vi "table line to assembly.vi"(11 "ItemNames":string[](array[string])) -> (3 "assembly definition":T1)   [LabVIEW 2013, in "EthernetIP editor node.lvclass"]
uses:
  EthernetIP editor node.lvclass
  configuration/assembly definition.ctl
  configuration/assembly type.ctl
  <vilib>/NI/Tag Bus/tag/Data Type.ctl
  configuration/EthernetIP configuration.lvclass
  <vilib>/NI/Tag Bus/tag/tag descriptor.lvclass
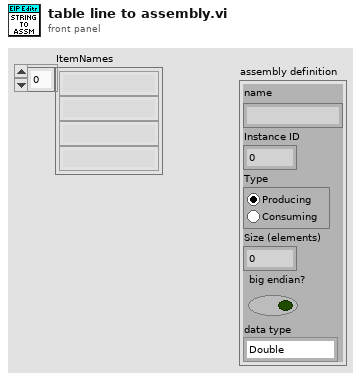
[diagram p1: front panel]
types:
  T1 = typedef "EthernetIP configuration.lvclass/assembly definition.ctl" = cluster{"name":string, "Instance ID":u32, "Type":T2, "Size (elements)":u32, "big endian?":bool, "data type":T3}
  T2 = typedef "EthernetIP configuration.lvclass/assembly type.ctl" = enum32{"Producing", "Consuming"}
  T3 = typedef "tag bus.lvlib/tag descriptor.lvclass/Data Type.ctl" = enum16{"Double", "Single", "I64", "I32", "I16", "I8", "U64", "U32", "U16", "U8", "Boolean", "String", "Array of Double", "Array of Single", "Array of I64", "Array of I32", "Array of I16", "Array of I8", "Array of U64", "Array of U32", "Array of U16", "Array of U8", "Array of Boolean", "Array of String"}
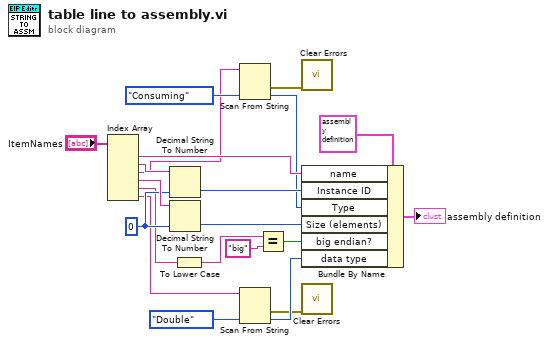
[diagram p0: block diagram]
diagram:
  w13 = u32 0 ("default (0 I32)")
  n1 = Index Array(array="ItemNames") -> (element #1=w18:string, element #2=w17:string, element #3=w9:string, element #4=w16:string, element #5=w8:string, element #6=w1:string)  [unwired: 6 in]
  n2 = Decimal String To Number(string=w17, default (0L)=w13) -> (number=w14:u32)  [unwired: 1 in, 1 out]
  n3 = Decimal String To Number(string=w16, default (0L)=w13) -> (number=w15:u32)  [unwired: 1 in, 1 out]
  n4 = To Lower Case(string=w8) -> (all lower case string=w5:string)
  n5 = Scan From String(input string=w9, default 1=assembly_type."Consuming" ("Type")) -> (error out=w12:errorcluster, output 1=w11:T2)  [unwired: 3 in, 2 out]
  n6 = Scan From String(input string=w1, default 1=Data_Type."Double" ("data type")) -> (error out=w2:errorcluster, output 1=w3:T3)  [unwired: 3 in, 2 out]
  n7 = Equal?(x=w5, y="big") -> (x = y?=w6:bool)
  n8 = call <vilib>:"Clear Errors.vi"("error in (no error)"=w12) -> ()  [unwired: 6 in, 1 out]
  n9 = Bundle By Name(cluster=T1 {"name"="", "Instance ID"=100, "Type"=enum."Producing", "Size (elements)"=32, "big endian?"=FALSE, "data type"=enum."Double"} ("assembly definition"), "name"=w18, "Instance ID"=w14, "Type"=w11, "Size (elements)"=w15, "big endian?"=w6, "data type"=w3) -> (→"assembly definition":T1)
  n10 = call <vilib>:"Clear Errors.vi"("error in (no error)"=w2) -> ()  [unwired: 6 in, 1 out]
